vi "TestSquareRoot.vi"(8 "error in (no error)":errorcluster) -> (0 "error out":errorcluster)   [LabVIEW 2016, in "SimpleCalculatorTests.lvlib"]
uses:
  SimpleCalculatorTests.lvlib
  APIs/Stimulus/KeyBoardSimulation/typedef/VirtualKey.ctl
  APIs/Stimulus/KeyBoardSimulation/typedef/Action.ctl
  APIs/Stimulus/ControlValue/SetValueAuto.vi
  APIs/Stimulus/KeyBoardSimulation/KeyboardSimulationCore.vi
  APIs/Stimulus/VI/CloseVI.vi
  APIs/Assert/AssertVI/Exec/AssertVIExecIdle.vi
  Drona.lvlib
  <vilib>/addons/_JKI Toolkits/Caraya/classes/Test/Test.lvclass
  <vilib>/SLL Toolkit/SLL Debug/SLL Debug.lvlib
  APIs/Stimulus/KeyBoardSimulation/KeyboardSimulation.lvlib
  APIs/Stimulus/ControlValue/ControlValue.lvlib
  APIs/Stimulus/VI/VI.lvlib
  APIs/Assert/AssertVI/AssertVI.lvlib
panel:
  # "Drona Test Square Root"
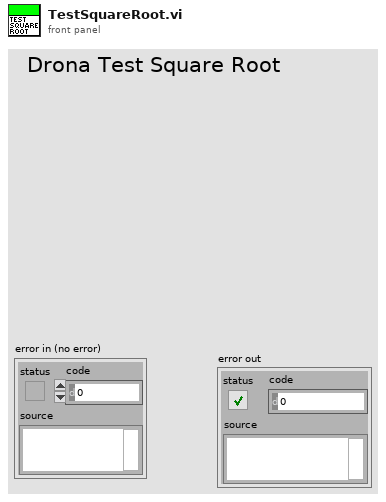
[diagram p1: front panel]
types:
  T1 = typedef "Drona.lvlib/KeyboardSimulation.lvlib/VirtualKey.ctl" = u8
  T2 = typedef "Drona.lvlib/KeyboardSimulation.lvlib/Action.ctl" = enum16{"Press", "Up", "Down"}
  T3 = cluster{"Key":T1, "Action":T2, "Delay (ms)":u32}[]
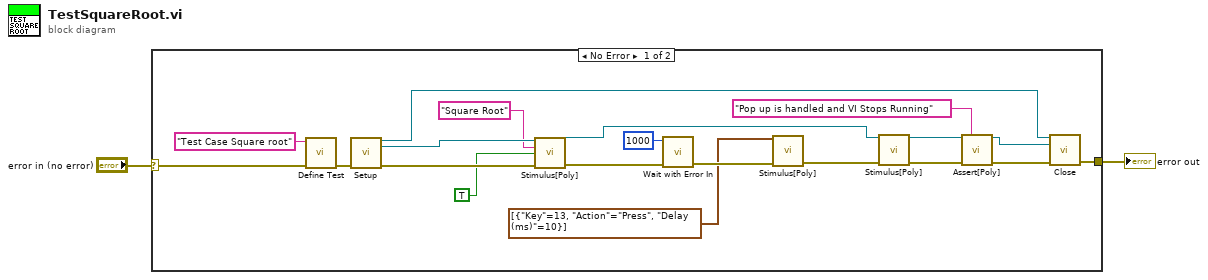
[diagram p0: block diagram]
diagram:
  n1 = case shown="No Error" "error in (no error)" {
    selector: "error in (no error)" -> [w13 w23]
    tunnel: [w9 w23] -> w1
    frame No Error {
      n2 = call <vilib>:"Define Test.vi"("error in (no error)"=w13, "Label (VI Title)"="Test Case Square root") -> ("error out"=w22:errorcluster)  [unwired: 8 in, 1 out]
      n3 = call "Setup.vi"("error in"=w22) -> ("Application Ref"=w10:refnum<vi>, "VI Reference Out"=w19:refnum<vi>, "error out"=w20:errorcluster)  [unwired: 12 in]
      n4 = call-poly "Stimulus[Poly].vi"("VI Reference In"=w19, "Control Path"="Square Root", "Value (Signaling)"=TRUE, "error in"=w20) -> ("VI Reference Out"=w11:refnum<vi>, "error out"=w16:errorcluster)  [unwired: 10 in]
      n5 = call <vilib>:"Wait with Error In.vi"("error in (no error)"=w16, "milliseconds to wait"=u32 1000) -> ("error out"=w14:errorcluster)  [unwired: 9 in]
      n6 = call-poly "Stimulus[Poly].vi"("Key Array"=T3 [{"Key"=13, "Action"=enum."Press", "Delay (ms)"=10}], "error in"=w14) -> ("error out"=w12:errorcluster)  [unwired: 13 in]
      n7 = call-poly "Stimulus[Poly].vi"("VI Reference In"=w11, "error in"=w12) -> ("VI Reference Out"=w7:refnum<vi>, "error out"=w8:errorcluster)  [unwired: 12 in]
      n8 = call-poly "Assert[Poly].vi"("VI Reference In"=w7, "Test Label"="Pop up is handled and VI Stops Running", "Error In"=w8) -> ("VI Reference Out"=w4:refnum<vi>, "Error Out"=w5:errorcluster)  [unwired: 10 in, 1 out]
      n9 = call "Close.vi"("Application Ref"=w10, "VI Reference"=w4, "error in"=w5) -> ("error out"=w9:errorcluster)  [unwired: 12 in]
    }
    frame Error {
    }
  }
  "error out" <- w1
